vi "Tags_Parse.vi"(0 "Words":i32[](array[numeric])) -> (1 "Right Step":i32, 2 "Left Step":i32, 3 "Home Step":i32, 4 "Right Count":i32, 5 "Left Count":i32, 6 "Cycles":i32, 7 "Alarm Code":i32, 8 "PLC Beat":i32, 9 "X":bool[](array[boolean]), 10 "Y":bool[](array[boolean]), 11 "Auto":bool, 12 "Manual":bool, 13 "Homed":bool, 14 "Alarm":bool, 15 "E-Stop":bool, 16 "Cycle Stop":bool, 17 "Connected":bool)   [LabVIEW 2018]
doc: "Use this template to build a VI to use as a subVI."
panel:
  # "說明：把 44 個字拆成各項狀態。0～41 ＝ D200～D241，\n42 ＝ M200～M205，43 ＝ 連線旗標。"
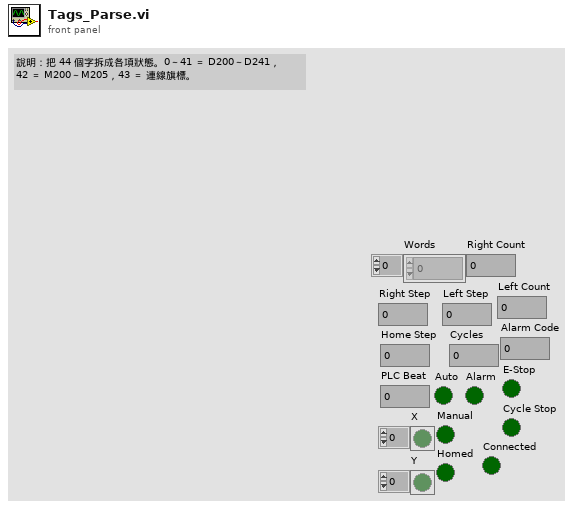
[diagram p1: front panel]
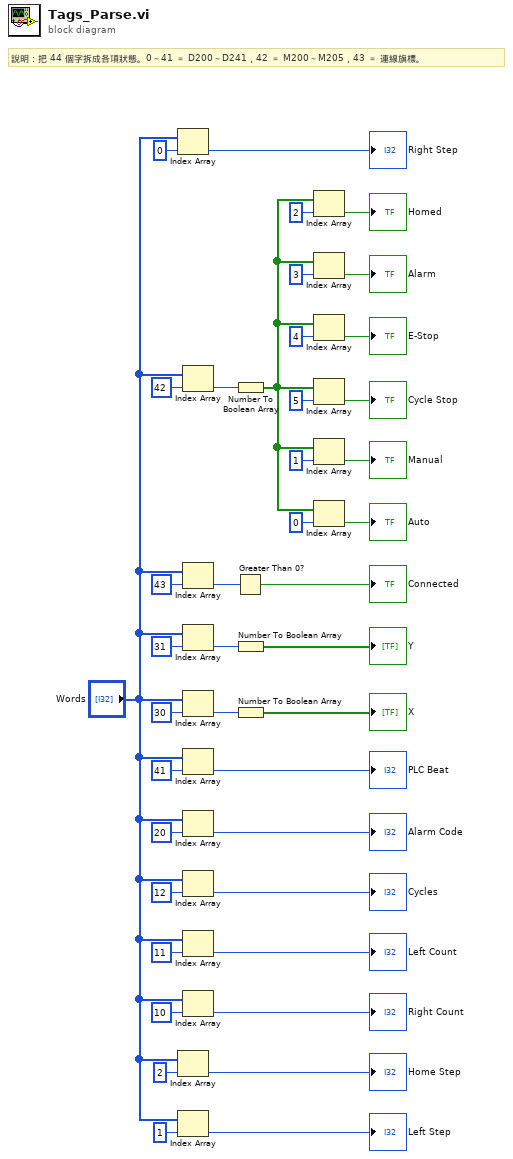
[diagram p0: block diagram]
diagram:
  # "說明：把 44 個字拆成各項狀態。0～41 ＝ D200～D241，42 ＝ M200～M205，43 ＝ 連線旗標。"
  n1 = Index Array(array="Words", index=0) -> (element=→"Right Step":i32)
  n2 = Index Array(array="Words", index=2) -> (element=→"Home Step":i32)
  n3 = Index Array(array="Words", index=1) -> (element=→"Left Step":i32)
  n4 = Index Array(array="Words", index=42) -> (element=w17:i32)
  n5 = Index Array(array="Words", index=43) -> (element=w2:i32)
  n6 = Index Array(array="Words", index=31) -> (element=w20:i32)
  n7 = Index Array(array="Words", index=30) -> (element=w23:i32)
  n8 = Index Array(array="Words", index=41) -> (element=→"PLC Beat":i32)
  n9 = Index Array(array="Words", index=20) -> (element=→"Alarm Code":i32)
  n10 = Index Array(array="Words", index=12) -> (element=→"Cycles":i32)
  n11 = Index Array(array="Words", index=11) -> (element=→"Left Count":i32)
  n12 = Index Array(array="Words", index=10) -> (element=→"Right Count":i32)
  n13 = Greater Than 0?(x=w2) -> (x > 0?=→"Connected":bool)
  n14 = Number To Boolean Array(number=w17) -> (Boolean array=w16:bool[])
  n15 = Number To Boolean Array(number=w20) -> (Boolean array=→"Y":bool[])
  n16 = Number To Boolean Array(number=w23) -> (Boolean array=→"X":bool[])
  n17 = Index Array(array=w16, index=2) -> (element=→"Homed":bool)
  n18 = Index Array(array=w16, index=3) -> (element=→"Alarm":bool)
  n19 = Index Array(array=w16, index=4) -> (element=→"E-Stop":bool)
  n20 = Index Array(array=w16, index=5) -> (element=→"Cycle Stop":bool)
  n21 = Index Array(array=w16, index=1) -> (element=→"Manual":bool)
  n22 = Index Array(array=w16, index=0) -> (element=→"Auto":bool)
